vi "Scheduler_Join_Branches.vi"(8 "error in (no error)":errorcluster={"status"=FALSE, "code"=0, "source"="\"\""}, 10 "group policy":string, 11 "Branch statuses":string) -> (0 "error out":errorcluster={"status"=FALSE, "code"=0, "source"="\"\""}, 2 "status ok":bool, 3 "Join outcome":string)   [LabVIEW 2026]
doc: "INTENT: Apply parallel join policy. LOGIC: Wait All/Selected/First Complete semantics; on declared fault preempt all; cancel unused branches safely."
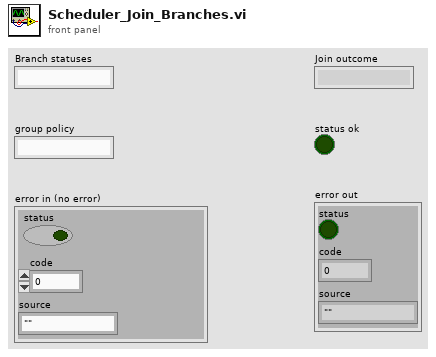
[diagram p1: front panel]
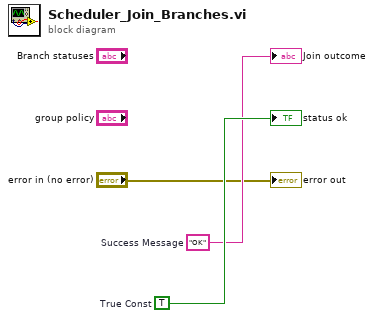
[diagram p0: block diagram]
diagram:
  w3 = TRUE  # True Const
  w2 = "OK"  # Success Message
  "Join outcome" <- w2
  "status ok" <- w3
  "error out" <- "error in (no error)"
